vi "Apply Package Name.vi"(8 "error in":errorcluster, 10 "package name":string, 11 "message metadata in":T1[](array[typedef])) -> (0 "error out":errorcluster, 3 "message metadata out":T1[](array[typedef]))   [LabVIEW 2019, in "grpc-lvsupport.lvlib"]
uses:
  grpc-lvsupport.lvlib
  typeDefs/Message Metadata.ctl
  typeDefs/Message Element Metadata.ctl
  typeDefs/Message Element Type.ctl
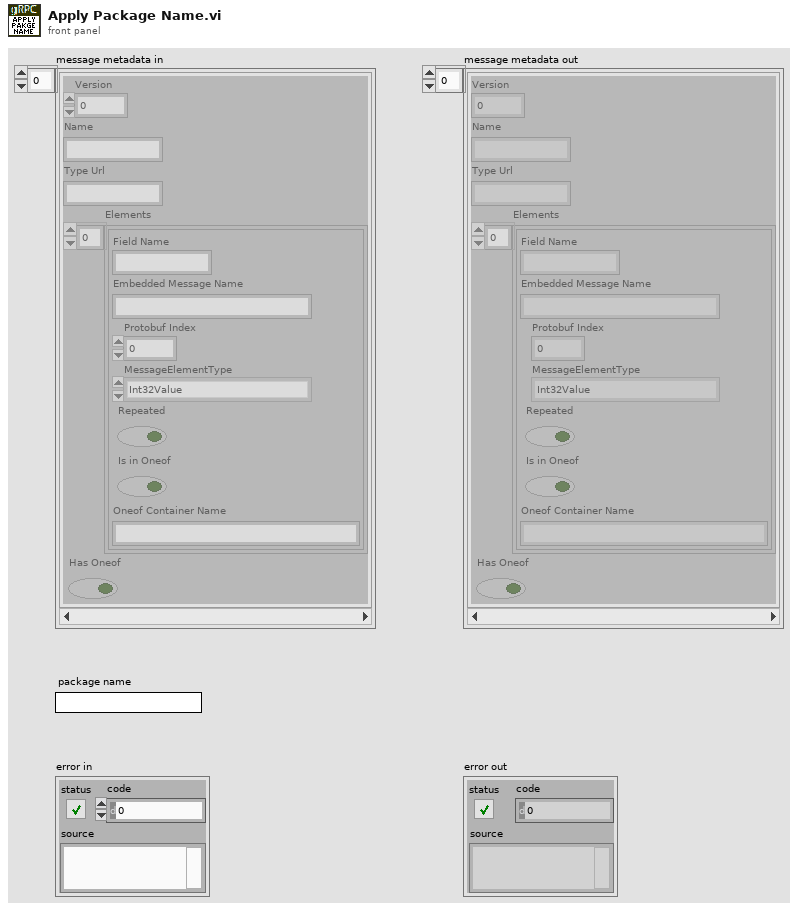
[diagram p1: front panel]
types:
  T1 = typedef "grpc-lvsupport.lvlib/Message Metadata.ctl" = cluster{"Version":i32, "Name":string, "Type Url":string, "Elements":T2[], "Has Oneof":bool}
  T2 = typedef "grpc-lvsupport.lvlib/Message Element Metadata.ctl" = cluster{"Field Name":string, "Embedded Message Name":string, "Protobuf Index":i32, "MessageElementType":T3, "Repeated":bool, "Is in Oneof":bool, "Oneof Container Name":string}
  T3 = typedef "grpc-lvsupport.lvlib/Message Element Type.ctl" = enum32{"Int32Value", "FloatValue", "DoubleValue", "BoolValue", "StringValue", "MessageValue", "Int64Value", "UInt32Value", "UInt64Value", "EnumValue", "Bytes", "Fixed64", "Fixed32", "SFixed64", "SFixed32", "SInt64", "SInt32"}
  T4 = typedef "grpc-lvsupport.lvlib/Well Known Types.ctl" = enum32{"None", "Double2DArray", "String2DArray"}
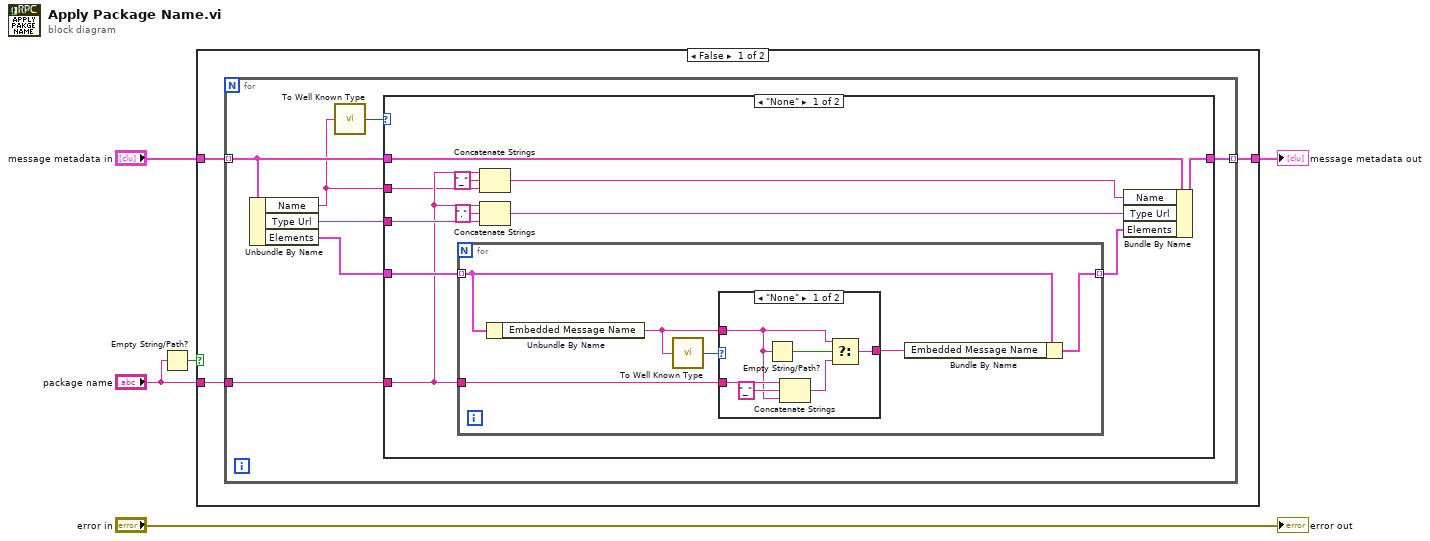
[diagram p0: block diagram]
diagram:
  n1 = Empty String/Path?(string/path="package name") -> (empty?=w1:bool)
  n2 = case shown="False" w1 {
    tunnel: "message metadata in" -> [w8 w41]
    tunnel: [w7 w41] -> w3
    tunnel: "package name" -> [w6 _]
    frame False {
      n3 = for {
        tunnel: w8 -> [w13] mode=indexing
        tunnel: w6 -> [w11]
        tunnel: [w12] -> w7 mode=indexing
        n4 = Unbundle By Name(w13) -> ("Name"=w10:string, "Type Url"=w14:string, "Elements"=w15:T2[])
        n5 = call "To Well Known Type.vi"("message name"=w10) -> ("well known type"=w9:T4)
        n6 = case shown="\"None\"" w9 {
          tunnel: w15 -> [w26 _]
          tunnel: w14 -> [w23 _]
          tunnel: w13 -> [w22 w40]
          tunnel: [w19 w40] -> w12
          tunnel: w11 -> [w17 _]
          tunnel: w10 -> [w16 _]
          frame "None" {
            n7 = for {
              tunnel: w26 -> [w32] mode=indexing
              tunnel: [w30] -> w18 mode=indexing
              tunnel: w17 -> [w29]
              n8 = Unbundle By Name(w32) -> ("Embedded Message Name"=w28:string)
              n9 = call "To Well Known Type.vi"("message name"=w28) -> ("well known type"=w27:T4)
              n10 = case shown="\"None\"" w27 {
                tunnel: [w35 w39] -> w31
                tunnel: w29 -> [w34 _]
                tunnel: w28 -> [w33 w39]
                frame "None" {
                  n11 = Empty String/Path?(string/path=w33) -> (empty?=w36:bool)
                  n12 = Concatenate Strings(w34, "_" ("string"), w33) -> (w37:string)
                  n13 = Select(t=w33, s=w36, f=w37) -> (s? t:f=w35:string)
                }
                frame Default {
                }
              }
              n14 = Bundle By Name(cluster=w32, "Embedded Message Name"=w31) -> (w30:T2)
            }
            n15 = Concatenate Strings(w17, "_" ("string"), w16) -> (w21:string)
            n16 = Concatenate Strings(w17, "." ("string"), w23) -> (w20:string)
            n17 = Bundle By Name(cluster=w22, "Name"=w21, "Type Url"=w20, "Elements"=w18) -> (w19:T1)
          }
          frame Default {
          }
        }
      }
    }
    frame True {
    }
  }
  "message metadata out" <- w3
  "error out" <- "error in"
